vi "SC Open Project File.vi"(8 "error in (no error)":errorcluster, 9 "path":path) -> (0 "error out":errorcluster)   [LabVIEW 2023]
doc: "Opens a LabVIEW project (or other LabVIEW file) the way File >> Open does, so its window appears."
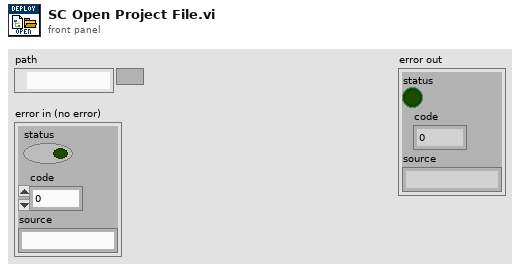
[diagram p1: front panel]
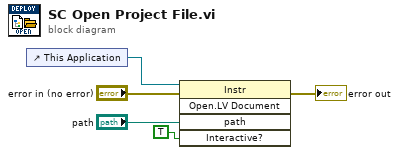
[diagram p0: block diagram]
diagram:
  n1 = control-ref of="This Application"() -> (w5:refnum<vi>)
  n2 = invoke class="Instr" method="Open.LV Document"(reference=w5, error in="error in (no error)", "path"="path", "Interactive?"=TRUE) -> (error out=→"error out":errorcluster)  [unwired: 1 in, 4 out]
